vi "VIH Debug Flag Container.vi"(7 "cmd (get)":enum16{"get", "set"}(ring), 11 "Debug Mode in":bool) -> (3 "Debug Mode":bool)   [LabVIEW 2014]
doc: "::: VI Helpeks :::\nCopyright (c) 2000-2026 Konstantin Shifershteyn. All rights reserved."
panel:
  # "VI Helpeks\nCopyright (c) 2012-2026 Konstantin Shifershteyn"
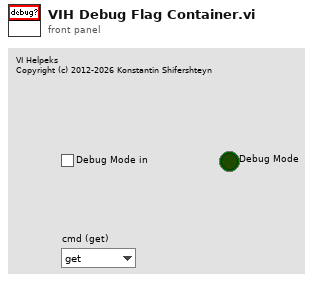
[diagram p1: front panel]
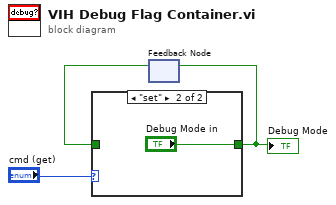
[diagram p0: block diagram]
diagram:
  n1 = feedback #1() -> (w2:bool)  [unwired: 1 in]
  n2 = case shown="\"set\"" "cmd (get)" {
    tunnel: [w4 "Debug Mode in"] -> w1
    tunnel: w2 -> [w4 _]
    frame "get" {
    }
    frame "set" {
    }
  }
  "Debug Mode" <- w1
  n3 = feedback-in #1(w1) -> ()
